vi "Test Insert sweepTable.vi"(8 "error in (no error)":errorcluster) -> (0 "error out":errorcluster)   [LabVIEW 2019, in "Tests.Instrument.Lockin.lvlib"]
uses:
  Tests.Instrument.Lockin.lvlib
  src/Instrument.Lockin/Instrument.Lockin.lvclass
  src/Lockin.Typedefs/Sweep/Sweep.Pattern--Enum.ctl
  src/Lockin.Typedefs/Lockin.Typedefs.lvlib
  src/Lockin.Typedefs/Sweep/Sweep.Channel--Cluster.ctl
  src/Lockin.Typedefs/Sweep/Sweep.Channel--Cluster--Array.ctl
  src/Lockin.Typedefs/Sweep/Sweep.Configuration--Cluster.ctl
  src/Lockin.Typedefs/API/Lockin.setSweep_Table--cluster.ctl
  <vilib>/addons/_JKI Toolkits/Caraya/classes/Test/Test.lvclass
  <vilib>/addons/_JKI Toolkits/Caraya/classes/Assert/Assert.lvclass
  <vilib>/addons/_JKI Toolkits/Caraya/classes/Assert/Assert True.vi
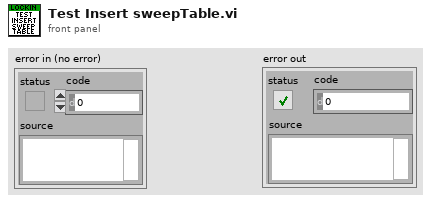
[diagram p1: front panel]
types:
  T1 = typedef "Lockin.Typedefs.lvlib/Sweep.Configuration--Cluster.ctl" = cluster{"initialWaitTime":dbl, "sweepTime":dbl, "returnToStart":bool, "sweepChannels":T2}
  T2 = typedef "Lockin.Typedefs.lvlib/Sweep.Channel--Cluster--Array.ctl" = T3[]
  T3 = typedef "Lockin.Typedefs.lvlib/Sweep.Channel--Cluster.ctl" = cluster{"Enable?":bool, "Channel":i32, "Start":dbl, "End":dbl, "Pattern":T4, "Table":dbl[]}
  T4 = typedef "Lockin.Typedefs.lvlib/Sweep.Pattern--Enum.ctl" = enum16{"Ramp /", "Ramp /\\", "Smooth Ramp _/", "Smooth Ramp _/\\_", "Table"}
  T5 = typedef "Lockin.Typedefs.lvlib/Lockin.setSweep_Table--cluster.ctl" = cluster{"Channel":i32, "Table":dbl[]}
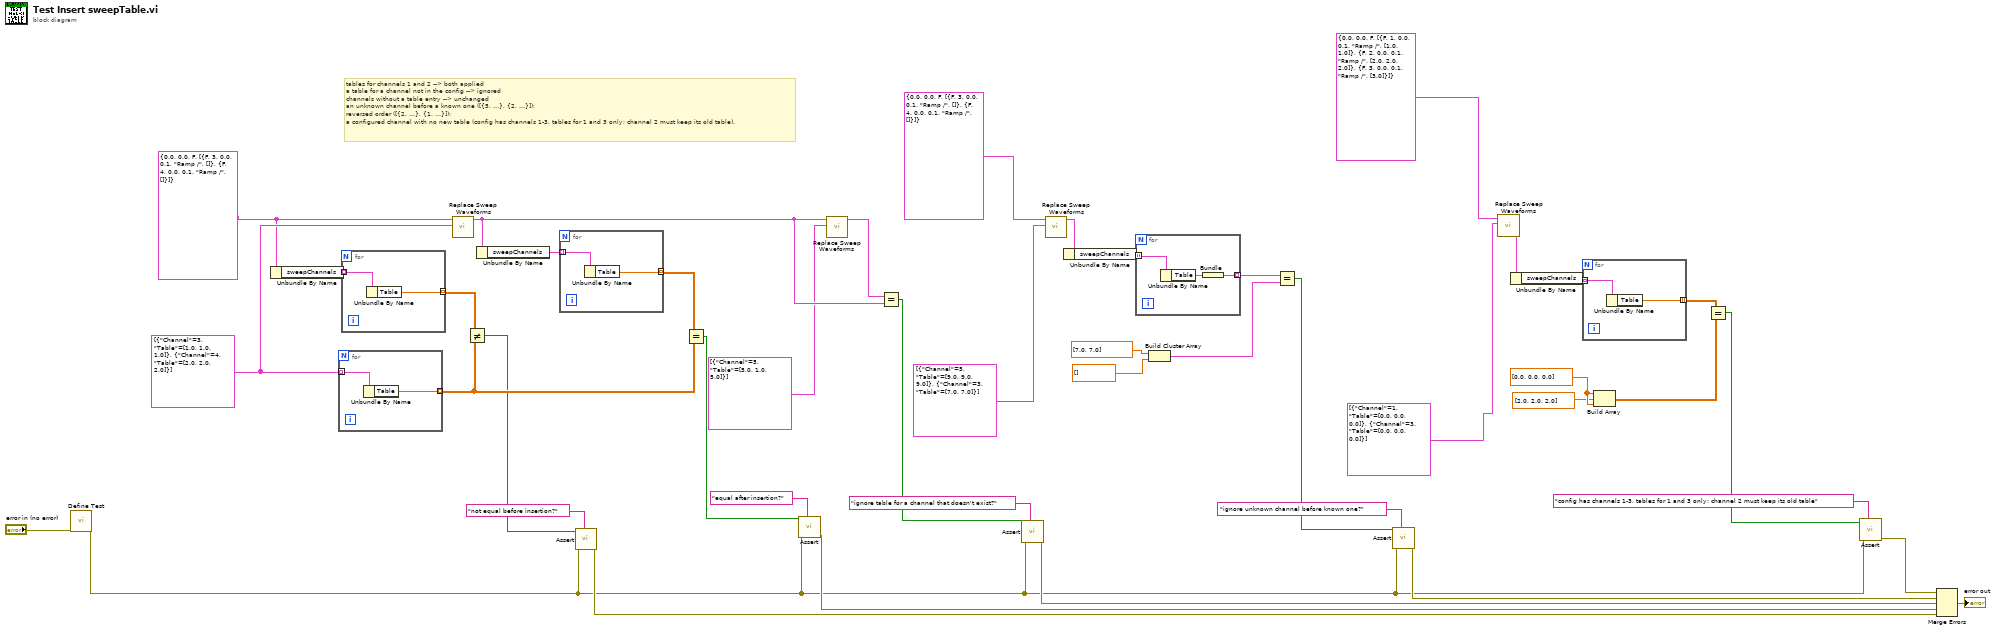
[diagram p0: block diagram]
diagram:
  w25 = T5[] [{"Channel"=3, "Table"=[1.0, 1.0, 1.0]}, {"Channel"=4, "Table"=[2.0, 2.0, 2.0]}] ("new Tables")
  w24 = T1 {"initialWaitTime"=0.0, "sweepTime"=0.0, "returnToStart"=FALSE, "sweepChannels"=[{"Enable?"=FALSE, "Channel"=3, "Start"=0.0, "End"=0.1, "Pattern"=enum."Ramp /", "Table"=[]}, {"Enable?"=FALSE, "Channel"=4, "Start"=0.0, "End"=0.1, "Pattern"=enum."Ramp /", "Table"=[]}]} ("Sweep in")
  w35 = dbl[] [0.0, 0.0, 0.0] ("Table")
  # "tables for channels 1 and 2 --> both applied\na table for a channel not in the config --> ignored\nchannels without a table entry --> unchanged\nan unknown channel before a known one ([{5, …}, {2, …}]);\nreversed order ([{2, …}, {1, …}]);\na configured channel with no new table (config has channels 1-3, tables for 1 and 3 only; channel 2 must keep its old table)."
  n1 = call <vilib>:"Define Test.vi"("error in (no error)"="error in (no error)") -> ("error out"=w3:errorcluster)  [unwired: 9 in, 1 out]
  n2 = Unbundle By Name(w24) -> ("sweepChannels"=w42:T2)
  n3 = for {
    tunnel: w25 -> [w46] mode=indexing
    tunnel: [w45] -> w40 mode=indexing
    n4 = Unbundle By Name(w46) -> ("Table"=w45:dbl[])
  }
  n5 = for {
    tunnel: w42 -> [w48] mode=indexing
    tunnel: [w47] -> w41 mode=indexing
    n6 = Unbundle By Name(w48) -> ("Table"=w47:dbl[])
  }
  n7 = call "Replace Sweep Waveforms.vi"("new Tables"=w25, "Sweep in"=w24) -> ("Sweep out"=w39:T1)  [unwired: 9 in]
  n8 = Not Equal?(x=w41, y=w40) -> (x != y?=w18:bool)
  n9 = Unbundle By Name(w39) -> ("sweepChannels"=w44:T2)
  n10 = for {
    tunnel: w44 -> [w50] mode=indexing
    tunnel: [w49] -> w43 mode=indexing
    n11 = Unbundle By Name(w50) -> ("Table"=w49:dbl[])
  }
  n12 = call-poly <vilib>:"Assert.vi"("Label"="not equal before insertion?", "error in (no error)"=w3, "True?"=w18) -> ("error out"=w4:errorcluster)  [unwired: 7 in, 1 out]
  n13 = Equal?(x=w43, y=w40) -> (x = y?=w12:bool)
  n14 = call-poly <vilib>:"Assert.vi"("Label"="equal after insertion?", "error in (no error)"=w3, "True?"=w12) -> ("error out"=w5:errorcluster)  [unwired: 7 in, 1 out]
  n15 = call "Replace Sweep Waveforms.vi"("new Tables"=T5[] [{"Channel"=5, "Table"=[5.0, 1.0, 5.0]}], "Sweep in"=w39) -> ("Sweep out"=w38:T1)  [unwired: 9 in]
  n16 = Equal?(x=w38, y=w39) -> (x = y?=w11:bool)
  n17 = call-poly <vilib>:"Assert.vi"("Label"="ignore table for a channel that doesn't exist?", "error in (no error)"=w3, "True?"=w11) -> ("error out"=w6:errorcluster)  [unwired: 7 in, 1 out]
  n18 = call "Replace Sweep Waveforms.vi"("new Tables"=T5[] [{"Channel"=5, "Table"=[9.0, 9.0, 9.0]}, {"Channel"=3, "Table"=[7.0, 7.0]}], "Sweep in"=T1 {"initialWaitTime"=0.0, "sweepTime"=0.0, "returnToStart"=FALSE, "sweepChannels"=[{"Enable?"=FALSE, "Channel"=3, "Start"=0.0, "End"=0.1, "Pattern"=enum."Ramp /", "Table"=[]}, {"Enable?"=FALSE, "Channel"=4, "Start"=0.0, "End"=0.1, "Pattern"=enum."Ramp /", "Table"=[]}]}) -> ("Sweep out"=w30:T1)  [unwired: 9 in]
  n19 = Unbundle By Name(w30) -> ("sweepChannels"=w31:T2)
  n20 = for {
    tunnel: w31 -> [w53] mode=indexing
    tunnel: [w51] -> w29 mode=indexing
    n21 = Unbundle By Name(w53) -> ("Table"=w52:dbl[])
    n22 = Bundle("Table"=w52) -> (w51:cluster{"Table":dbl[]})  [unwired: 1 in]
  }
  n23 = Build Cluster Array(dbl[] [7.0, 7.0] ("Table"), dbl[] [] ("Table")) -> (w26:cluster{"Table":dbl[]}[])
  n24 = Equal?(x=w29, y=w26) -> (x = y?=w10:bool)
  n25 = call-poly <vilib>:"Assert.vi"("Label"="ignore unknown channel before known one?", "error in (no error)"=w3, "True?"=w10) -> ("error out"=w7:errorcluster)  [unwired: 7 in, 1 out]
  n26 = call "Replace Sweep Waveforms.vi"("new Tables"=T5[] [{"Channel"=1, "Table"=[0.0, 0.0, 0.0]}, {"Channel"=3, "Table"=[0.0, 0.0, 0.0]}], "Sweep in"=T1 {"initialWaitTime"=0.0, "sweepTime"=0.0, "returnToStart"=FALSE, "sweepChannels"=[{"Enable?"=FALSE, "Channel"=1, "Start"=0.0, "End"=0.1, "Pattern"=enum."Ramp /", "Table"=[1.0, 1.0]}, {"Enable?"=FALSE, "Channel"=2, "Start"=0.0, "End"=0.1, "Pattern"=enum."Ramp /", "Table"=[2.0, 2.0, 2.0]}, {"Enable?"=FALSE, "Channel"=3, "Start"=0.0, "End"=0.1, "Pattern"=enum."Ramp /", "Table"=[3.0]}]}) -> ("Sweep out"=w37:T1)  [unwired: 9 in]
  n27 = Unbundle By Name(w37) -> ("sweepChannels"=w36:T2)
  n28 = for {
    tunnel: w36 -> [w55] mode=indexing
    tunnel: [w54] -> w33 mode=indexing
    n29 = Unbundle By Name(w55) -> ("Table"=w54:dbl[])
  }
  n30 = Build Array(w35, dbl[] [2.0, 2.0, 2.0] ("Table"), w35) -> (w32:dbl[][])
  n31 = Equal?(x=w33, y=w32) -> (x = y?=w9:bool)
  n32 = call-poly <vilib>:"Assert.vi"("Label"="config has channels 1-3, tables for 1 and 3 only; channel 2 must keep its old table", "error in (no error)"=w3, "True?"=w9) -> ("error out"=w8:errorcluster)  [unwired: 7 in, 1 out]
  n33 = Merge Errors(w8, w7, w6, w5, w4) -> (→"error out":errorcluster)
